vi "Load Default Configuration.vi"(8 "error in (no error)":errorcluster, 11 "CIFPlugin in":refnum<class "CAN_Reader_CANsub_Plugin.lvclass">) -> (0 "error out":errorcluster, 3 "CIFPlugin out":refnum<class "CAN_Reader_CANsub_Plugin.lvclass">)   [LabVIEW 2021, in "CAN_Reader_CANsub_Plugin.lvclass"]
uses:
  CAN_Reader_CANsub_Plugin.lvclass
  CAN_Reader_CANsub_Plugin.lvclass/CAN_Reader_CANsub_Plugin.ctl
  <vilib>/CIF Foundation/CIF Core/CIFCore/Common/Typedef/Common Plugin Configuration.ctl
  <vilib>/CIF Foundation/CIF Core/CIFCore/Common/CIFCoreCommon.lvlib
  <vilib>/CIF Foundation/CIF Core/CIFCore/Class/CIFCorePlugin.lvclass
  C:/Program Files/National Instruments/LabVIEW 2021/vi.lib/CIF Foundation/CIF Core/CIFCore/Class/CIFCorePlugin.lvclass
  <vilib>/CIF Foundation/CIF Core/CIFCore/Common/Typedef/External Clock Config.ctl
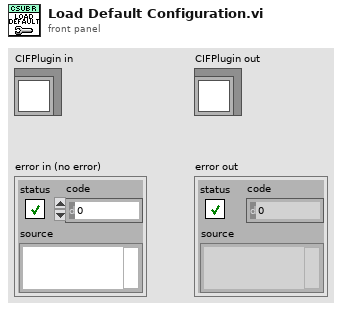
[diagram p1: front panel]
types:
  T1 = typedef "CIFCoreCommon.lvlib/Common Plugin Configuration.ctl" = cluster{"Period (s)":dbl, "Offset (us)":i32, "Priority":i32, "Processor":i32, "External Clock":T2}
  T2 = typedef "CIFCoreCommon.lvlib/External Clock Config.ctl" = cluster{"ClockID":u8, "Clock Name":string, "Publish Clock":bool, "Convert Data Timestamps":bool, "Plugin Timing Source":bool}
  T3 = typedef "CAN_Reader_CANsub_Common.lvlib/Configuration.ctl" = cluster{"Common":T1, "RX Interface":string, "Port Configuration":T4, "Timeout (ms)":i32, "Frames to read":i32, "Filter":T7}
  T4 = typedef "CAN_RW_CORE.lvclass/CAN Port Configuration.ctl" = cluster{"Mode":T5, "Baud Rate":u64, "Temination On":bool, "Subordinate":bool, "Echo TX":bool, "FD Config":T6}
  T5 = typedef "CAN_RW_CORE.lvclass/CAN Mode.ctl" = enum16{"CAN 2.0", "CAN FD"}
  T6 = typedef "CAN_RW_CORE.lvclass/FD Config.ctl" = cluster{"FD Baud Rate":u64, "ISO Mode":bool, "BRS Enabled":bool}
  T7 = typedef "CAN_RW_CORE.lvclass/CAN Filter.ctl" = cluster{"Allow List (ID)":u32[], "Deny List (ID)":u32[]}
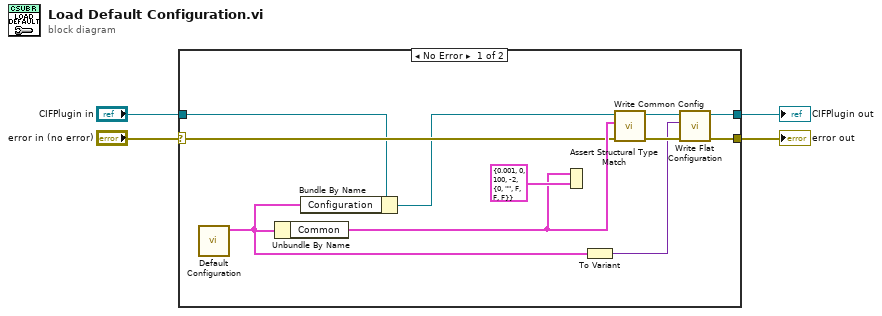
[diagram p0: block diagram]
diagram:
  n1 = case shown="No Error" "error in (no error)" {
    selector: "error in (no error)" -> [w8 w16]
    tunnel: "CIFPlugin in" -> [w7 w17]
    tunnel: [w11 w17] -> w1
    tunnel: [w10 w16] -> w3
    frame No Error {
      n2 = call "Default Configuration.vi"() -> ("Default Configuration"=w6:T3)  [unwired: 11 in]
      n3 = Unbundle By Name(w6) -> ("Common"=w14:T1)
      n4 = Bundle By Name(cluster=w7, "Configuration"=w6) -> (w5:refnum<class "CAN_Reader_CANsub_Plugin.lvclass">)
      n5 = Assert Structural Type Match(0:T1 {"Period (s)"=0.001, "Offset (us)"=0, "Priority"=100, "Processor"=-2, "External Clock"={"ClockID"=0, "Clock Name"="", "Publish Clock"=FALSE, "Convert Data Timestamps"=FALSE, "Plugin Timing Source"=FALSE}} ("Common"), 1:w14) -> ()
      n6 = To Variant(anything=w6) -> (Variant=w9:variant)
      n7 = call <vilib>:"Write Common Config.vi"("error in (no error)"=w8, "Common"=w14, "CIFTemplateNode in"=w5) -> ("error out"=w12:errorcluster, "CIFTemplateNode out"=w13:refnum<class "CAN_Reader_CANsub_Plugin.lvclass">)  [unwired: 7 in]
      n8 = call <vilib>:"Write Flat Configuration.vi"("error in (no error)"=w12, "Configuration"=w9, "CIFTemplateNode in"=w13) -> ("error out"=w10:errorcluster, "CIFTemplateNode out"=w11:refnum<class "CAN_Reader_CANsub_Plugin.lvclass">)  [unwired: 7 in]
    }
    frame Error {
    }
  }
  "error out" <- w3
  "CIFPlugin out" <- w1
